vi "Replace Dependency.vi"(6 "New SubVI":path, 8 "error in":errorcluster, 9 "SubVI":string, 10 "VI Path":path, 11 "LV File Creator in":refnum<class "LV File Creator.lvclass">) -> (0 "error out":errorcluster, 3 "LV File Creator out":refnum<class "LV File Creator.lvclass">)   [LabVIEW 2026, in "LV File Creator.lvclass"]
doc: "This VI will open a reference to the provided VI path, traverse objects and replace the specified SubVI by the new SubVI."
uses:
  LV File Creator.lvclass
  LV File Creator.lvclass/LV File Creator.ctl
  <vilib>/Utility/traverseref.llb/TRef TravTarget.ctl
  Interfaces/ILogger/ILogger Messages/Log Msg/Log Msg.lvclass/Log Msg.ctl
  <vilib>/ActorFramework/Message Enqueuer/Message Enqueuer.lvclass/Message Enqueuer.ctl
  <vilib>/ActorFramework/Message Enqueuer/Enqueue.vi
  Interfaces/ILogger/ILogger Messages/Log Msg/Log Msg.lvclass
  <userlib>/_OpenG.lib/file/file.llb/Strip Path Extension - Path__ogtk.vi
  <vilib>/ActorFramework/Message Priority Queue/Priority Enqueue.vi
  <userlib>/_OpenG.lib/file/file.llb/openg_file.lvlib
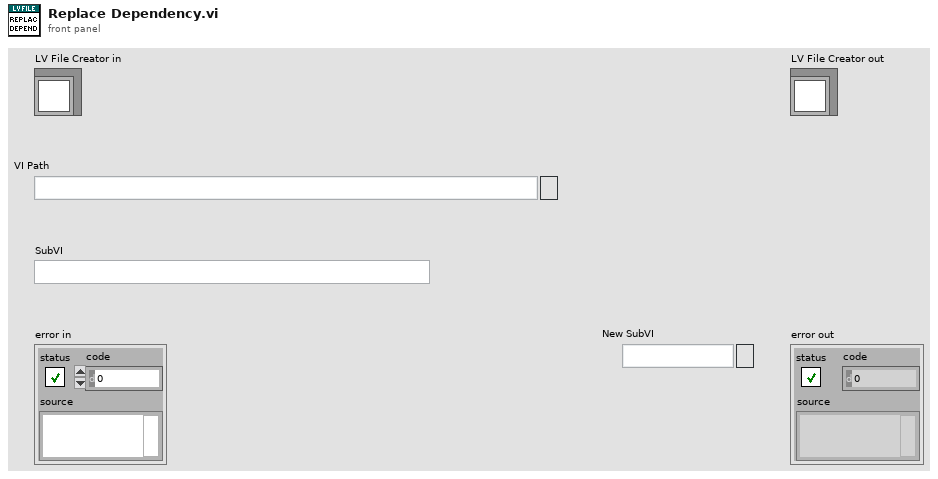
[diagram p1: front panel]
types:
  T1 = typedef "TRef TravTarget.ctl" = enum16{"FP", "BD", "Other"}
  T2 = typedef "Log Entry--cluster.ctl" = cluster{"Time":timestamp, "Message":string}
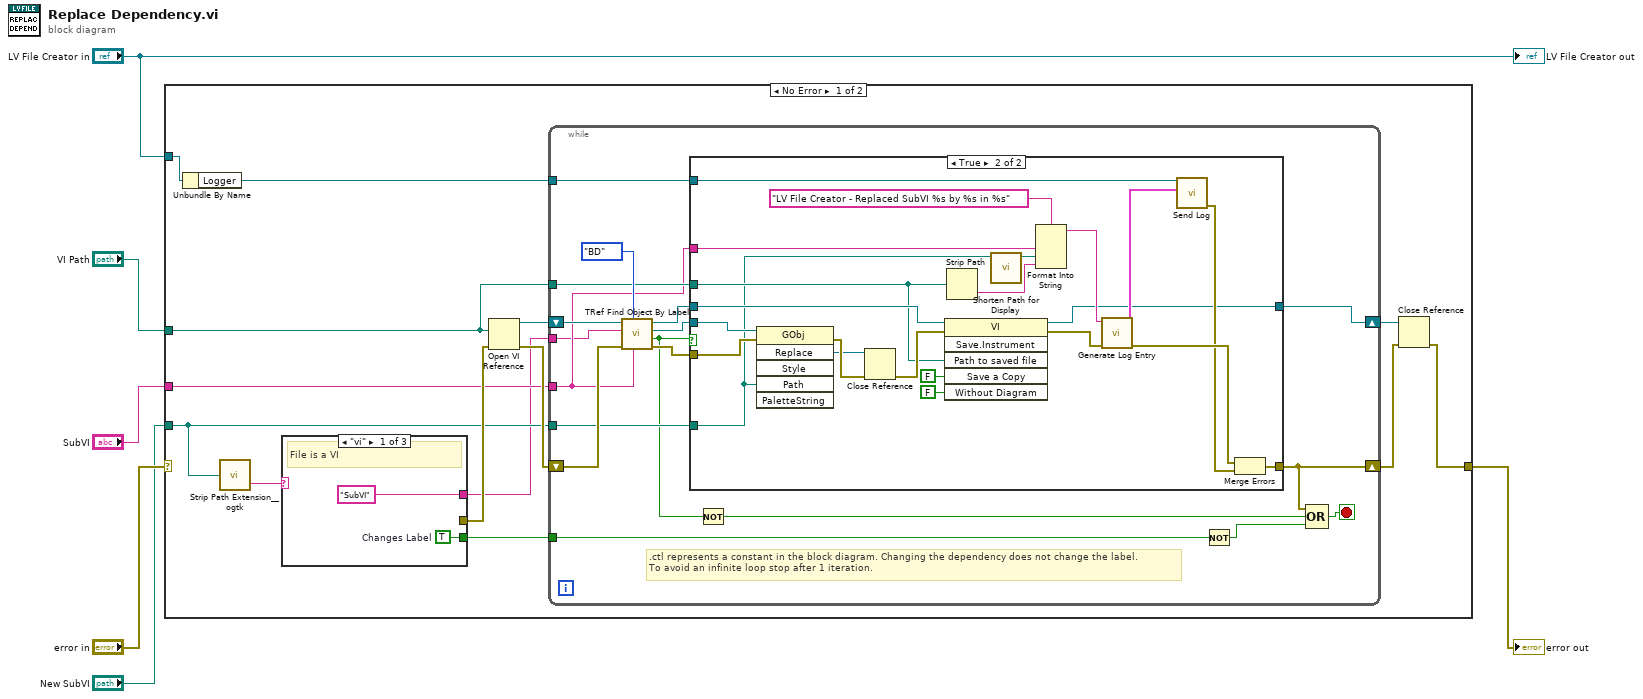
[diagram p0: block diagram]
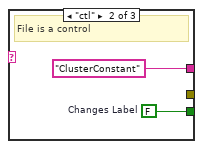
[diagram p3: hidden frame]
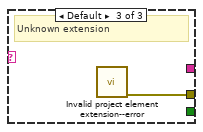
[diagram p4: hidden frame]
diagram:
  n1 = case shown="No Error" "error in" {
    selector: "error in" -> [_ w68]
    tunnel: [w17 w68] -> w5
    tunnel: "VI Path" -> [w13 _]
    tunnel: "SubVI" -> [w12 _]
    tunnel: "New SubVI" -> [w10 _]
    tunnel: "LV File Creator in" -> [w15 _]
    frame No Error {
      n2 = Unbundle By Name(w15) -> ("Logger"=w14:refnum<class "Message Enqueuer.lvclass">)
      n3 = call-poly <userlib>:"Strip Path Extension__ogtk.vi"("path"=w10) -> ("extension"=w11:string)  [unwired: 1 out]
      n4 = case shown="\"vi\"" w11 {
        tunnel: [_ _ w67] -> w19
        tunnel: ["SubVI" ("Class Name") "ClusterConstant" ("Type") _] -> w9
        tunnel: [w63 w65 _] -> w7
        frame "vi" {
          w63 = TRUE  # Changes Label
          # "File is a VI"
        }
        frame "ctl" {
          w65 = FALSE  # Changes Label
          # "File is a control"
        }
        frame Default {
          # "Unknown extension"
          n5 = call "Invalid project element extension--error.vi"() -> ("error out"=w67:errorcluster)  [unwired: 11 in]
        }
      }
      n6 = Open VI Reference(vi path=w13, error in (no error)=w19) -> (vi reference=w16:refnum<vi>, error out=w20:errorcluster)  [unwired: 4 in]
      n7 = while {
        tunnel: w14 -> [w31]
        tunnel: w13 -> [w30]
        tunnel: w12 -> [w29]
        tunnel: w10 -> [w28]
        tunnel: w9 -> [w27]
        shift-right: [w36] -> w18
        shift-left: w20 -> [w38]
        shift-right: [w23] -> w8
        shift-left: w16 -> [w35]
        tunnel: w7 -> [w22]
        stop <- w24 stop-if-true
        # ".ctl represents a constant in the block diagram. Changing the dependency does not change the label.\nTo avoid an infinite loop stop after 1 iteration."
        n8 = call <vilib>:"TRef Find Object By Label.vi"("Label"=w29, "Traverse Target"=TRef_TravTarget."BD", "error in (no error)"=w38, "Class Name"=w27, "VI Ref"=w35) -> ("error out"=w37:errorcluster, "Found?"=w26:bool, "Found Obj Ref"=w33:refnum<vi>, "dup VI Ref"=w32:refnum<vi>)  [unwired: 3 in]
        n9 = case shown="True" w26 {
          tunnel: w37 -> [w40 w62]
          tunnel: [w40 w58] -> w36
          tunnel: w33 -> [_ w55]
          tunnel: w32 -> [w39 w53]
          tunnel: w31 -> [_ w50]
          tunnel: w30 -> [_ w46]
          tunnel: w29 -> [_ w44]
          tunnel: w28 -> [_ w43]
          tunnel: [w39 w41] -> w23
          frame False {
          }
          frame True {
            n10 = invoke on="Invoke Node" class="GObj" method="Replace"(reference=w55, error in=w62, "Path"=w43) -> (error out=w61:errorcluster, "Replace"=w54:refnum<vi>)  [unwired: 3 in, 4 out]
            n11 = Close Reference(reference=w54, error in (no error)=w61) -> (error out=w60:errorcluster)
            n12 = invoke on="Invoke Node" class="VI" method="Save.Instrument"(reference=w53, error in=w60, "Path to saved file"=w46, "Save a Copy"=FALSE, "Without Diagram"=FALSE) -> (reference out=w41:refnum<vi>, error out=w56:errorcluster)  [unwired: 1 in, 4 out]
            n13 = Strip Path(path=w46) -> (name=w45:string)  [unwired: 1 out]
            n14 = call "Shorten Path for Display.vi"("Path"=w43) -> ("Shortened Path"=w42:path)  [unwired: 10 in]
            n15 = Format Into String(format string="LV File Creator - Replaced SubVI %s by %s in %s", w44, w42, w45) -> (resulting string=w48:string)  [unwired: 2 in, 1 out]
            n16 = call "Generate Log Entry.vi"("error in"=w56, "Message"=w48) -> ("error out"=w59:errorcluster, "Log Entry"=w47:T2)  [unwired: 8 in]
            n17 = call "Send Log.vi"("Log Entry"=w47, "Message Enqueuer"=w50) -> ("error out"=w57:errorcluster)  [unwired: 8 in, 1 out]
            n18 = Merge Errors(w59, w57) -> (w58:errorcluster)
          }
        }
        n19 = Not(x=w26) -> (.not. x?=w25:bool)
        n20 = Not(x=w22) -> (.not. x?=w21:bool)
        n21 = Compound Arithmetic op=OR(w36, w25, w21) -> (w24:bool)
      }
      n22 = Close Reference(reference=w8, error in (no error)=w18) -> (error out=w17:errorcluster)
    }
    frame Error {
      # "Pass error without actions."
    }
  }
  "error out" <- w5
  "LV File Creator out" <- "LV File Creator in"
